vi "Should Send Progress.vi"(7 "cancelled?":bool, 8 "error in":errorcluster, 9 "streaming?":bool, 10 "last progress":dbl=nan, 11 "progress":dbl) -> (0 "error out":errorcluster, 3 "send?":bool)   [LabVIEW 2020, in "MCP Server.lvlib"]
doc: "Decides whether Report Progress.vi sends a notifications/progress event: TRUE when the call is streamed, not cancelled, error in carries no error, progress is a number, and progress is larger than the last progress sent (or nothing was sent yet: last progress NaN). Used by Report Progress.vi.\n\nerror in is passed through unchanged."
uses:
  MCP Server.lvlib
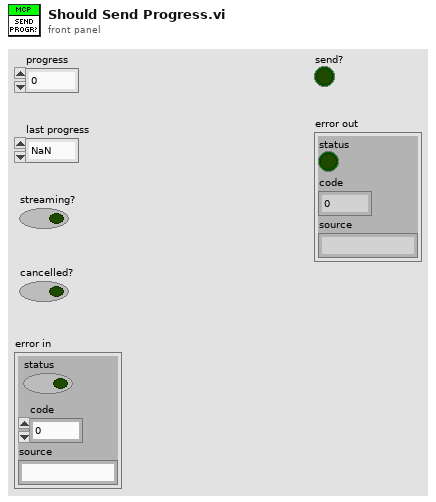
[diagram p1: front panel]
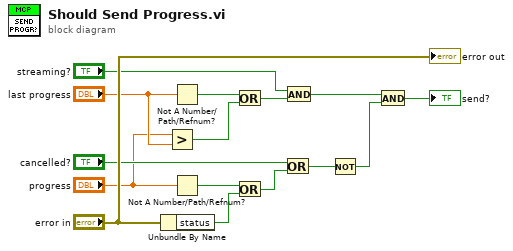
[diagram p0: block diagram]
diagram:
  n1 = Unbundle By Name("error in") -> ("status"=w10:bool)
  n2 = Greater?(x="progress", y="last progress") -> (0:w7:bool)
  n3 = Not A Number/Path/Refnum?(number/path/refnum="last progress") -> (NaN/Path/Refnum?=w6:bool)
  n4 = Not A Number/Path/Refnum?(number/path/refnum="progress") -> (NaN/Path/Refnum?=w9:bool)
  n5 = Or(x=w6, y=w7) -> (x .or. y?=w8:bool)
  n6 = Or(x=w9, y=w10) -> (x .or. y?=w11:bool)
  n7 = Or(x="cancelled?", y=w11) -> (x .or. y?=w12:bool)
  n8 = And(x="streaming?", y=w8) -> (x .and. y?=w14:bool)
  n9 = Not(x=w12) -> (.not. x?=w13:bool)
  n10 = And(x=w14, y=w13) -> (x .and. y?=→"send?":bool)
  "error out" <- "error in"
